vi "GetPID.vi"(8 "error in (no error)":errorcluster) -> (0 "error out":errorcluster, 3 "PID":i32)   [LabVIEW 2017]
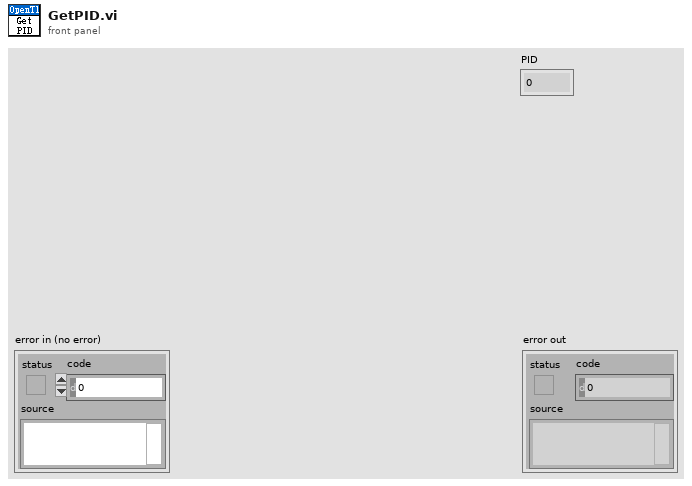
[diagram p1: front panel]
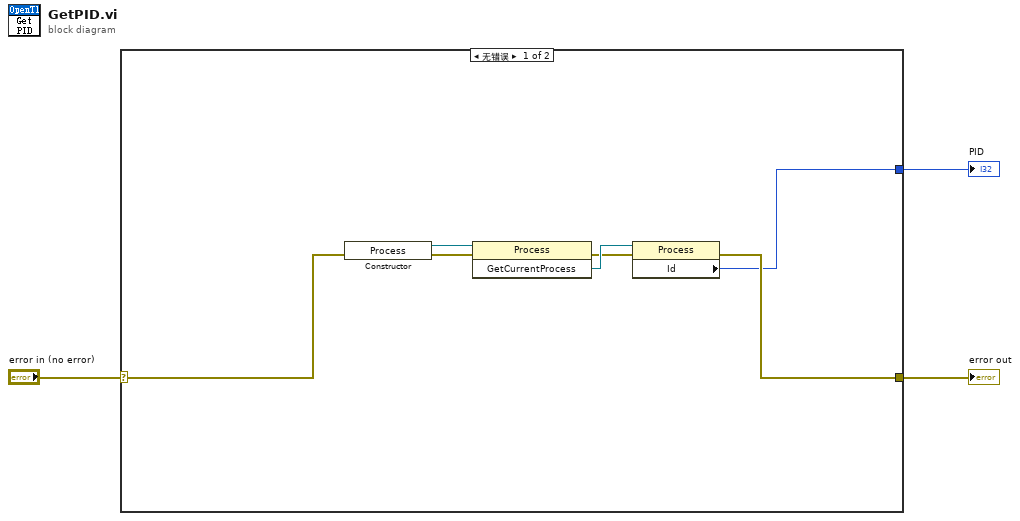
[diagram p0: block diagram]
diagram:
  n1 = case shown="无错误" "error in (no error)" {
    selector: "error in (no error)" -> [w6 w11]
    tunnel: [w5 w11] -> w2
    tunnel: [w4 _] -> w1
    frame No Error {
      n2 = constructor class="Process"(error in=w6) -> (reference out=w10:refnum<k24>, error out=w8:errorcluster)  [unwired: 2 in, 1 out]
      n3 = invoke on="调用节点" class="Process" method="GetCurrentProcess"(reference=w10, error in=w8) -> (error out=w7:errorcluster, "GetCurrentProcess"=w9:refnum<k24>)  [unwired: 1 in, 1 out]
      n4 = property on="属性节点" class="Process"(reference=w9, error in=w7) -> (error out=w5:errorcluster, "Id"=w4:i32)  [unwired: 1 out]
    }
    frame Error {
    }
  }
  "error out" <- w2
  "PID" <- w1
